vi "RDC-saltwater-read_parameter.vi"() -> (1 "Array":T1[](array[typedef]), 2 "map":map{u16, T1}(c390))   [LabVIEW 2020, in "RDC-Reflection_Data_Computation.lvlib"]
doc: "Parses the salt water parameter table stored in the VI into an array and a map keyed by temperature x10."
uses:
  RDC-Reflection_Data_Computation.lvlib
  RDC-saltwater-param.ctl
panel:
  out "string array":string[](array[string])
  out "array w/ subset deleted":string[](array[string])
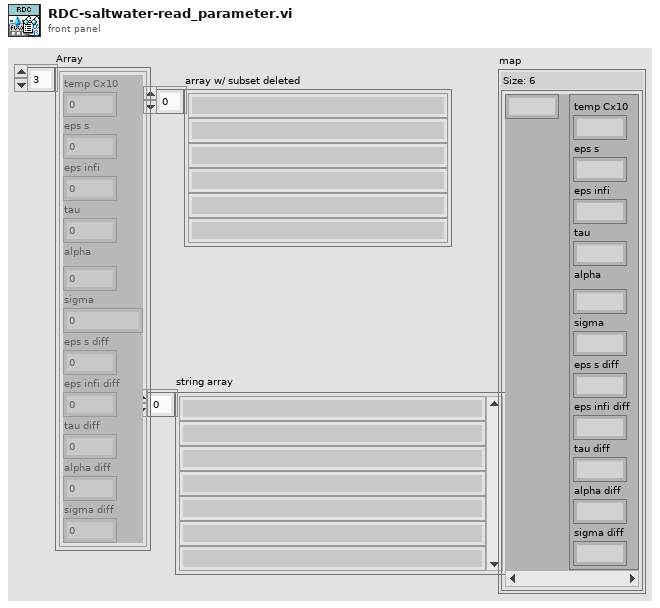
[diagram p1: front panel]
types:
  T1 = typedef "RDC-Reflection_Data_Computation.lvlib/RDC-saltwater-param.ctl" = cluster{"temp Cx10":u16, "eps s":dbl, "eps infi":dbl, "tau":dbl, "alpha":dbl, "sigma":dbl, "eps s diff":dbl, "eps infi diff":dbl, "tau diff":dbl, "alpha diff":dbl, "sigma diff":dbl}
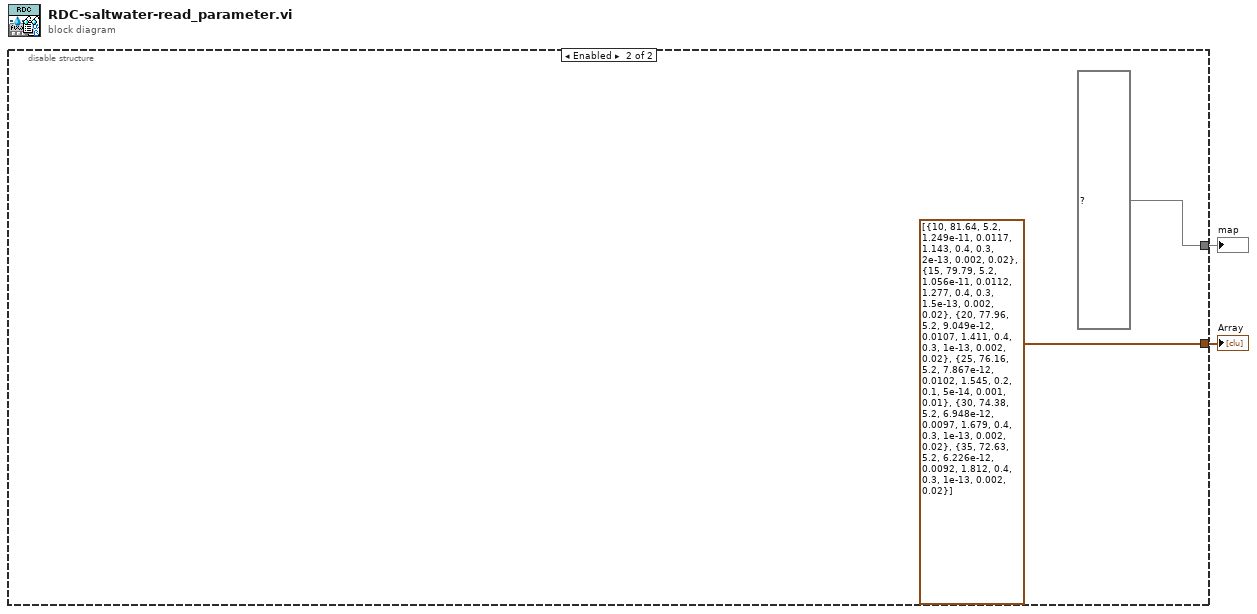
[diagram p0: block diagram]
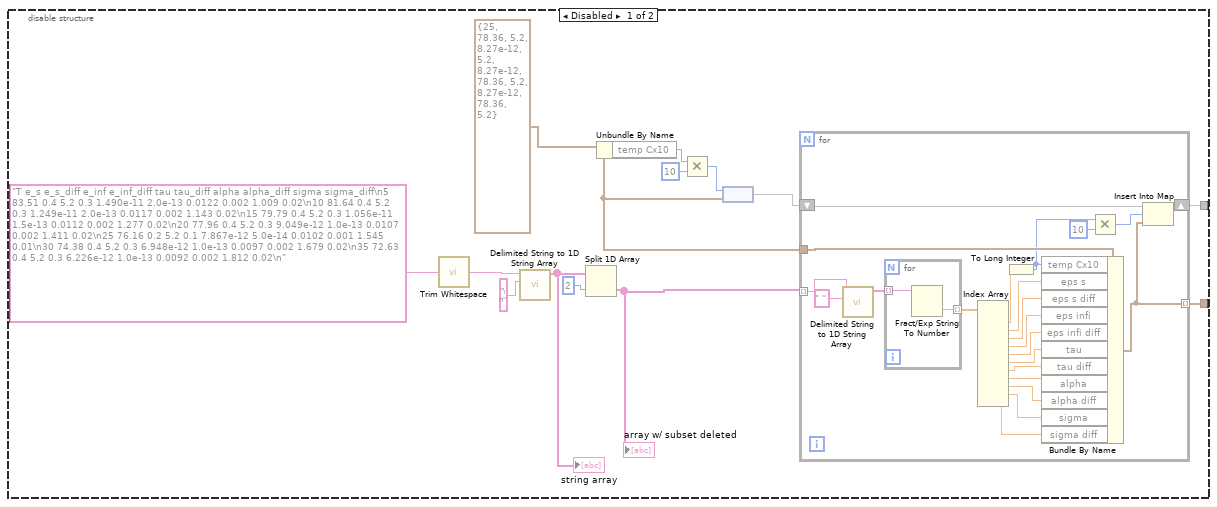
[diagram p2: hidden frame]
diagram:
  n1 = disable-structure shown="Enabled" {
    disable-tunnel: [w6 map{u16, T1} {100={"temp Cx10"=10, "eps s"=81.64, "eps infi"=5.2, "tau"=1.249e-11, "alpha"=0.0117, "sigma"=1.143, "eps s diff"=0.4, "eps infi diff"=0.3, "tau diff"=2e-13, "alpha diff"=0.002, "sigma diff"=0.02}, 150={"temp Cx10"=15, "eps s"=79.79, "eps infi"=5.2, "tau"=1.056e-11, "alpha"=0.0112, "sigma"=1.277, "eps s diff"=0.4, "eps infi diff"=0.3, "tau diff"=1.5e-13, "alpha diff"=0.002, "sigma diff"=0.02}, 200={"temp Cx10"=20, "eps s"=77.96, "eps infi"=5.2, "tau"=9.049e-12, "alpha"=0.0107, "sigma"=1.411, "eps s diff"=0.4, "eps infi diff"=0.3, "tau diff"=1e-13, "alpha diff"=0.002, "sigma diff"=0.02}, 250={"temp Cx10"=25, "eps s"=76.16, "eps infi"=5.2, "tau"=7.867e-12, "alpha"=0.0102, "sigma"=1.545, "eps s diff"=0.2, "eps infi diff"=0.1, "tau diff"=5e-14, "alpha diff"=0.001, "sigma diff"=0.01}, 300={"temp Cx10"=30, "eps s"=74.38, "eps infi"=5.2, "tau"=6.948e-12, "alpha"=0.0097, "sigma"=1.679, "eps s diff"=0.4, "eps infi diff"=0.3, "tau diff"=1e-13, "alpha diff"=0.002, "sigma diff"=0.02}, 350={"temp Cx10"=35, "eps s"=72.63, "eps infi"=5.2, "tau"=6.226e-12, "alpha"=0.0092, "sigma"=1.812, "eps s diff"=0.4, "eps infi diff"=0.3, "tau diff"=1e-13, "alpha diff"=0.002, "sigma diff"=0.02}} ("map 2")] -> w2
    disable-tunnel: [w5 T1[] [{"temp Cx10"=10, "eps s"=81.64, "eps infi"=5.2, "tau"=1.249e-11, "alpha"=0.0117, "sigma"=1.143, "eps s diff"=0.4, "eps infi diff"=0.3, "tau diff"=2e-13, "alpha diff"=0.002, "sigma diff"=0.02}, {"temp Cx10"=15, "eps s"=79.79, "eps infi"=5.2, "tau"=1.056e-11, "alpha"=0.0112, "sigma"=1.277, "eps s diff"=0.4, "eps infi diff"=0.3, "tau diff"=1.5e-13, "alpha diff"=0.002, "sigma diff"=0.02}, {"temp Cx10"=20, "eps s"=77.96, "eps infi"=5.2, "tau"=9.049e-12, "alpha"=0.0107, "sigma"=1.411, "eps s diff"=0.4, "eps infi diff"=0.3, "tau diff"=1e-13, "alpha diff"=0.002, "sigma diff"=0.02}, {"temp Cx10"=25, "eps s"=76.16, "eps infi"=5.2, "tau"=7.867e-12, "alpha"=0.0102, "sigma"=1.545, "eps s diff"=0.2, "eps infi diff"=0.1, "tau diff"=5e-14, "alpha diff"=0.001, "sigma diff"=0.01}, {"temp Cx10"=30, "eps s"=74.38, "eps infi"=5.2, "tau"=6.948e-12, "alpha"=0.0097, "sigma"=1.679, "eps s diff"=0.4, "eps infi diff"=0.3, "tau diff"=1e-13, "alpha diff"=0.002, "sigma diff"=0.02}, {"temp Cx10"=35, "eps s"=72.63, "eps infi"=5.2, "tau"=6.226e-12, "alpha"=0.0092, "sigma"=1.812, "eps s diff"=0.4, "eps infi diff"=0.3, "tau diff"=1e-13, "alpha diff"=0.002, "sigma diff"=0.02}] ("Array 2")] -> w1
    frame Disabled {
      w3 = T1 {"temp Cx10"=25, "eps s"=78.36, "eps infi"=5.2, "tau"=8.27e-12, "alpha"=5.2, "sigma"=8.27e-12, "eps s diff"=78.36, "eps infi diff"=5.2, "tau diff"=8.27e-12, "alpha diff"=78.36, "sigma diff"=5.2} ("water values")
      n2 = call <vilib>:"Trim Whitespace.vi"("string"="T e_s e_s_diff e_inf e_inf_diff tau tau_diff alpha alpha_diff sigma sigma_diff\n5 83.51 0.4 5.2 0.3 1.490e-11 2.0e-13 0.0122 0.002 1.009 0.02\n10 81.64 0.4 5.2 0.3 1.249e-11 2.0e-13 0.0117 0.002 1.143 0.02\n15 79.79 0.4 5.2 0.3 1.056e-11 1.5e-13 0.0112 0.002 1.277 0.02\n20 77.96 0.4 5.2 0.3 9.049e-12 1.0e-13 0.0107 0.002 1.411 0.02\n25 76.16 0.2 5.2 0.1 7.867e-12 5.0e-14 0.0102 0.001 1.545 0.01\n30 74.38 0.4 5.2 0.3 6.948e-12 1.0e-13 0.0097 0.002 1.679 0.02\n35 72.63 0.4 5.2 0.3 6.226e-12 1.0e-13 0.0092 0.002 1.812 0.02\n") -> ("trimmed string"=w4:string)  [unwired: 1 in]
      n3 = call <vilib>:"Delimited String to 1D String Array.vi"("delimiter"="\n", "delimited string"=w4) -> ("string array"=w13:string[])  [unwired: 9 in]
      "string array" <- w13
      n4 = Split 1D Array(array=w13, index=2) -> (second subarray=w12:string[])  [unwired: 1 out]
      "array w/ subset deleted" <- w12
      n5 = Unbundle By Name(w3) -> ("temp Cx10"=w10:u16)
      n6 = Multiply(x=w10, y=u16 10) -> (x*y=w7:u16)
      n7 = node(w7, w3) -> (w8:map{u16, T1})
      n8 = for {
        tunnel: w12 -> [w37] mode=indexing
        tunnel: w3 -> [w33]
        tunnel: [w20] -> w5 mode=indexing
        shift-right: [w24] -> w6
        shift-left: w8 -> [w25]
        n9 = call <vilib>:"Delimited String to 1D String Array.vi"("delimiter"=" ", "delimited string"=w37) -> ("string array"=w35:string[])  [unwired: 9 in]
        n10 = for {
          tunnel: w35 -> [w39] mode=indexing
          tunnel: [w38] -> w34 mode=indexing
          n11 = Fract/Exp String To Number(string=w39) -> (number=w38:dbl)  [unwired: 3 in, 1 out]
        }
        n12 = Index Array(array=w34) -> (element #1=w32:dbl, element #2=w31:dbl, element #3=w30:dbl, element #4=w29:dbl, element #5=w28:dbl, element #6=w27:dbl, element #7=w26:dbl, element #8=w19:dbl, element #9=w18:dbl, element #10=w17:dbl, element #11=w16:dbl)  [unwired: 11 in]
        n13 = To Long Integer(number=w32) -> (32bit integer=w22:i32)
        n14 = Bundle By Name(cluster=w33, "temp Cx10"=w22, "eps s"=w31, "eps s diff"=w30, "eps infi"=w29, "eps infi diff"=w28, "tau"=w27, "tau diff"=w26, "alpha"=w19, "alpha diff"=w18, "sigma"=w17, "sigma diff"=w16) -> (w20:T1)
        n15 = Multiply(x=w22, y=u16 10) -> (x*y=w21:i32)
        n16 = Insert Into Map(map in=w25, key=w21, value=w20) -> (map out=w24:map{u16, T1})  [unwired: 2 out]
      }
    }
    frame Enabled {
    }
  }
  "map" <- w2
  "Array" <- w1
